vi "Exo_5.2.vi"() -> ()   [LabVIEW 2012]
uses:
  <vilib>/Analysis/baseanly.llb/Mean (DBL).vi
  <vilib>/Analysis/NI_AALBase.lvlib
panel:
  out "Array":dbl[](array[numeric])
  out "mean":dbl format="%0.2f"
  in  "N 2":i32
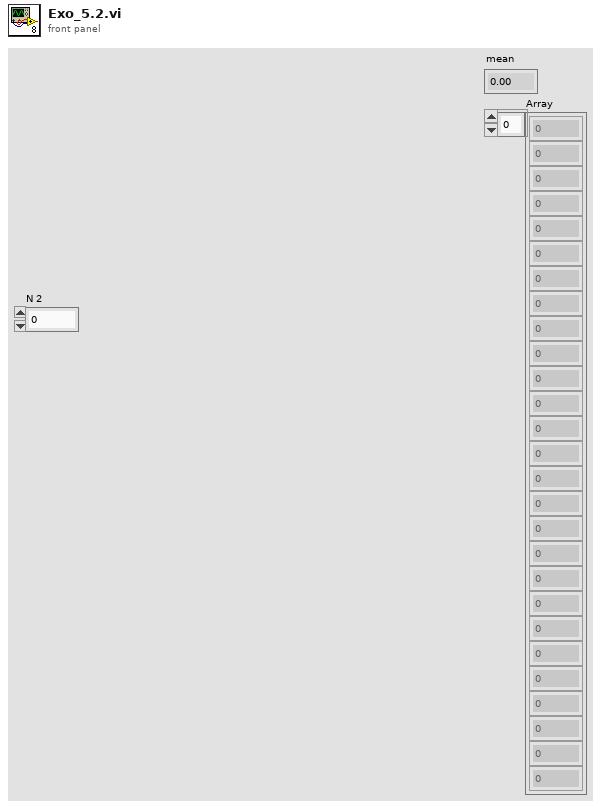
[diagram p1: front panel]
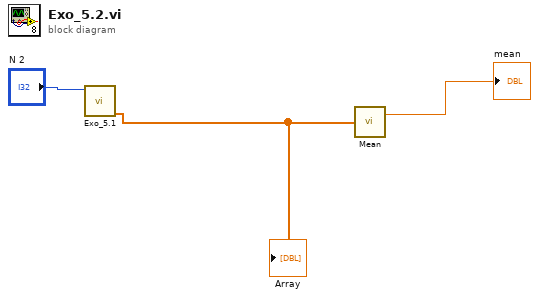
[diagram p0: block diagram]
diagram:
  n1 = call "Exo_5.1.vi"("N"="N 2") -> ("Array"=w2:dbl[])  [unwired: 10 in]
  "Array" <- w2
  n2 = call-poly <vilib>:"Mean.vi"("X"=w2) -> ("mean"=→"mean":dbl)  [unwired: 1 out]
